vi "DropVI_SimpleReconnectingPublisher.vi"() -> ()   [LabVIEW 2013, in "MQTT Client.lvlib"]
uses:
  MQTT Client.lvlib
  Client class/Client.lvclass/Client.ctl
  <vilib>/LabVIEW Open Source Project/MQTT Connection/MQTT_Base/Base Class/MQTT_Base.lvclass/MQTT_Base.ctl
  <vilib>/LabVIEW Open Source Project/MQTT Control Packets/Control Packets/PUBLISH/PUBLISH.lvclass
  Client class/Client.lvclass
  <vilib>/LabVIEW Open Source Project/MQTT Connection/MQTT_Base/Base Class/MQTT_Base.lvclass
  <vilib>/LabVIEW Open Source Project/Connection/Connection/Connection.lvclass
  <vilib>/LabVIEW Open Source Project/Connection/Connection.TCP/Connection.TCP.lvclass
  <vilib>/LabVIEW Open Source Project/Connection/Connection.LocalQueue/Connection.LocalQueue.lvclass
panel:
  out "Connected":bool
  out "last error":errorcluster
  out "Waveform Chart":dbl(graph)
  out "Published":bool
  in  "Stop Client":bool
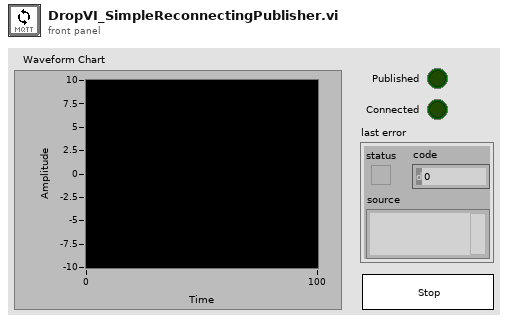
[diagram p1: front panel]
types:
  T1 = typedef "MQTT Client.lvlib/Client.lvclass/Public Events -- cluster.ctl" = cluster{"Connection Status":refnum<user-event>, "Connected":refnum<user-event>, "Application Message":refnum<user-event>}
  T2 = typedef "MQTT Base.lvlib/MQTT_Base.lvclass/Public Events -- cluster.ctl" = cluster{"Stop Event":refnum<user-event>, "Error Event":refnum<user-event>, "Inbound Message":refnum<user-event>}
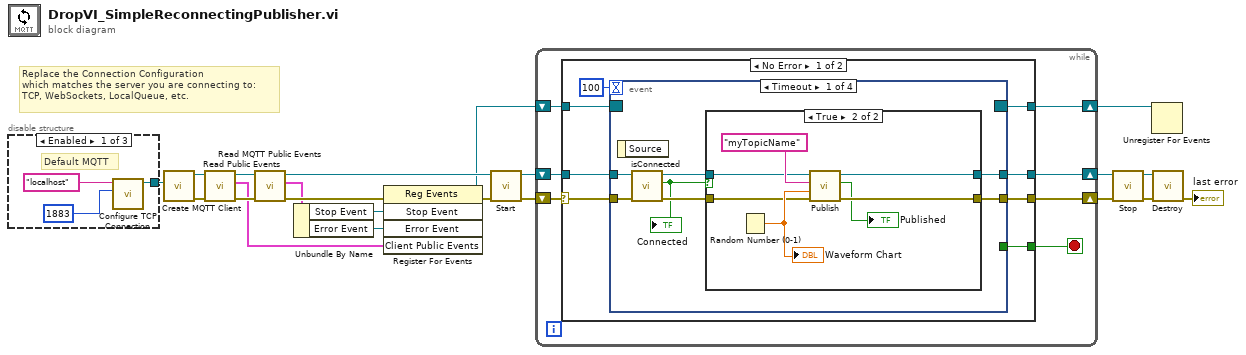
[diagram p0: block diagram]
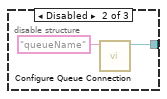
[diagram p2: hidden frame]
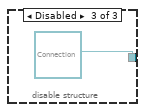
[diagram p3: hidden frame]
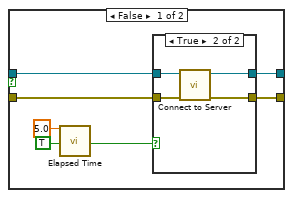
[diagram p4: hidden frame]
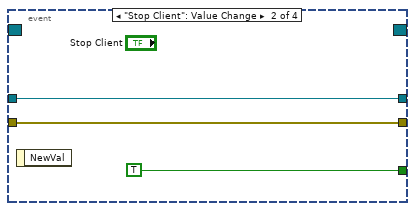
[diagram p6: hidden frame]
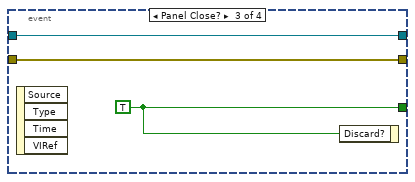
[diagram p7: hidden frame]
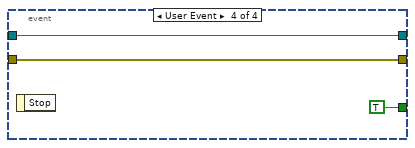
[diagram p8: hidden frame]
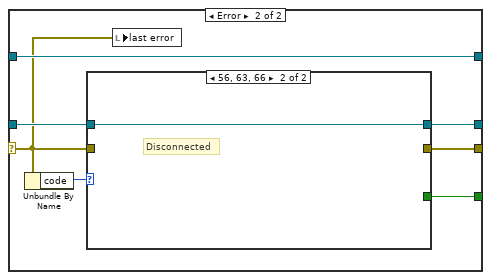
[diagram p9: hidden frame]
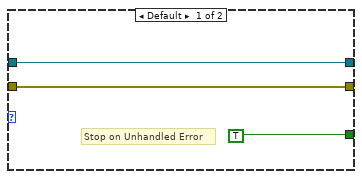
[diagram p10: hidden frame]
diagram:
  # "Replace the Connection Configuration\nwhich matches the server you are connecting to:\nTCP, WebSockets, LocalQueue, etc."
  n1 = disable-structure shown="Enabled" {
    disable-tunnel: [w23 w26 refnum<class "Connection.lvclass"> refnum ("Connection Configuration")] -> w1
    frame Enabled {
      # "Default MQTT"
      n2 = call <vilib>:"Configure TCP Connection.vi"("remote port (80)"=u16 1883, "address (localhost)"="localhost") -> ("Connection.TCP"=w23:refnum<class "Connection.TCP.lvclass">)  [unwired: 8 in, 1 out]
    }
    frame Disabled {
      n3 = call <vilib>:"Configure Queue Connection.vi"("Queue Name"="queueName") -> ("Connection.LocalQueue"=w26:refnum<class "Connection.LocalQueue.lvclass">)  [unwired: 9 in, 1 out]
    }
    frame Disabled {
    }
  }
  n4 = call "Create MQTT Client.vi"("Connection Configuration"=w1) -> ("error out"=w19:errorcluster, "Client out"=w21:refnum<class "Client.lvclass">)  [unwired: 9 in]
  n5 = call "Read Public Events.vi"("error in (no error)"=w19, "Client in"=w21) -> ("error out"=w18:errorcluster, "Client Public Events"=w16:T1, "Client out"=w20:refnum<class "Client.lvclass">)  [unwired: 7 in]
  n6 = call <vilib>:"Read MQTT Public Events.vi"("error in (no error)"=w18, "MQTT_Base in"=w20) -> ("error out"=w17:errorcluster, "MQTT Public Events"=w9:T2, "MQTT_Base out"=w14:refnum<class "Client.lvclass">)  [unwired: 7 in]
  n7 = Unbundle By Name(w9) -> ("Stop Event"=w11:refnum<user-event>, "Error Event"=w10:refnum<user-event>)
  n8 = register-events(error in=w17, w11, w10, w16) -> (reference out=w13:refnum<event-registration>, error out=w15:errorcluster)  [unwired: 1 in]
  n9 = call <vilib>:"Start.vi"("error in (no error)"=w15, "MQTT_Base in"=w14) -> ("error out"=w3:errorcluster, "MQTT_Base out"=w4:refnum<class "Client.lvclass">)  [unwired: 7 in, 1 out]
  n10 = while {
    shift-right: [w33] -> w12
    shift-left: w13 -> [w34]
    shift-right: [w30] -> w7
    shift-left: w4 -> [w31]
    shift-right: [w32] -> w5
    shift-left: w3 -> [w28]
    stop <- w29 stop-if-true
    n11 = case shown="No Error" w28 {
      selector: w28 -> [w35 w79]
      tunnel: w34 -> [w42 w85]
      tunnel: [w41 w85] -> w33
      tunnel: [w40 w81] -> w32
      tunnel: w31 -> [w38 w83]
      tunnel: [w37 w82] -> w30
      tunnel: [w36 w80] -> w29
      frame No Error {
        n12 = event shown="[0] Timeout" {
          selector: w42 -> [_ _ _ _]
          dyn-events: [_ _ _ _] -> w41
          timeout: 100 -> [_ _ _ _]
          tunnel: w35 -> [w45 w71 w73 w78]
          tunnel: [w48 w71 w73 w78] -> w40
          tunnel: [_ TRUE w75 TRUE] -> w36
          tunnel: w38 -> [w47 w72 w74 w76]
          tunnel: [w49 w72 w74 w76] -> w37
          event Timeout {
            n13 = event-data() -> ()  [unwired: 1 in, 1 out]
            n14 = call "isConnected.vi"("error in (no error)"=w45, "Client in"=w47) -> ("error out"=w44:errorcluster, "connected"=w43:bool, "Client out"=w46:refnum<class "Client.lvclass">)  [unwired: 7 in]
            "Connected" <- w43
            n15 = case shown="True" w43 {
              tunnel: [w55 w68] -> w49
              tunnel: [w53 w67] -> w48
              tunnel: w46 -> [w56 w64]
              tunnel: w44 -> [w54 w63]
              frame False {
                n16 = call "Elapsed Time"("Time Target (s)"=5.0, "Auto Reset"=TRUE) -> ("Time has Elapsed"=w52:bool)  [unwired: 10 in, 7 out]
                n17 = case shown="True" w52 {
                  tunnel: w56 -> [w58 w62]
                  tunnel: [w58 w61] -> w55
                  tunnel: w54 -> [w57 w60]
                  tunnel: [w57 w59] -> w53
                  frame False {
                  }
                  frame True {
                    n18 = call "Connect to Server.vi"("error in (no error)"=w60, "Client in"=w62) -> ("error out"=w59:errorcluster, "Client out"=w61:refnum<class "Client.lvclass">)  [unwired: 6 in, 2 out]
                  }
                }
              }
              frame True {
                n19 = Random Number (0-1)() -> (number: 0 to 1=w65:dbl)
                "Waveform Chart" <- w65
                n20 = call "Publish.vi"("error in (no error)"=w63, "Payload"=w65, "Topic Name (empty: Payload name)"="myTopicName", "Client in"=w64) -> ("error out"=w67:errorcluster, "Published"=→"Published":bool, "Client out"=w68:refnum<class "Client.lvclass">)  [unwired: 5 in]
              }
            }
          }
          event "Stop Client": Value Change {
            n21 = event-data() -> ()  [unwired: 1 in, 1 out]
          }
          event Panel Close? {
            w75 = TRUE
            n22 = event-data() -> ()  [unwired: 1 in, 4 out]
            n23 = event-data("Discard?"=w75) -> ()  [unwired: 1 in, 1 out]
          }
          event User Event {
            n24 = event-data() -> ()  [unwired: 1 in, 1 out]
          }
        }
      }
      frame Error {
        n25 = Unbundle By Name(w79) -> ("code"=w84:i32)
        n26 = case shown="56, 63, 66" w84 {
          tunnel: w83 -> [w88 w89]
          tunnel: [w88 w89] -> w82
          tunnel: w79 -> [w87 _]
          tunnel: [w87 _] -> w81
          tunnel: [TRUE _] -> w80
          frame Default {
            # "Stop on Unhandled Error"
          }
          frame 56, 63, 66 {
            # "Disconnected"
          }
        }
        n27 = local write "last error"(w79) -> ()
      }
    }
  }
  n28 = call <vilib>:"Stop.vi"("error in (no error)"=w5, "MQTT_Base in"=w7) -> ("error out"=w6:errorcluster, "MQTT_Base out"=w8:refnum<class "Client.lvclass">)  [unwired: 7 in, 1 out]
  n29 = Unregister For Events(event registration refnum=w12) -> ()  [unwired: 1 in, 1 out]
  n30 = call <vilib>:"Destroy.vi"("error in (no error)"=w6, "MQTT_Base in"=w8) -> ("error out"=→"last error":errorcluster)  [unwired: 8 in, 1 out]
